vi "Transport_Reconnect.vi"(8 "error in (no error)":errorcluster={"status"=FALSE, "code"=0, "source"="\"\""}, 10 "reconnection policy":string, 11 "Channel refs":string) -> (0 "error out":errorcluster={"status"=FALSE, "code"=0, "source"="\"\""}, 2 "status ok":bool, 3 "New connection or failure":string)   [LabVIEW 2026]
doc: "INTENT: Recover non-running communication session. LOGIC: Tear down broken refs, negotiate capabilities, reconcile run identity and report outstanding status."
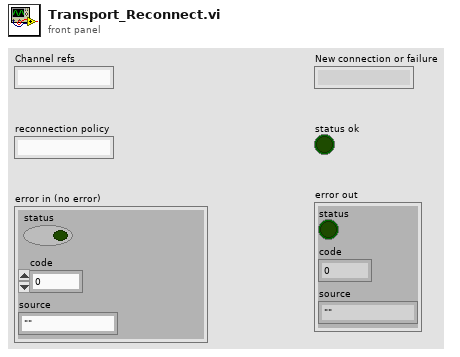
[diagram p1: front panel]
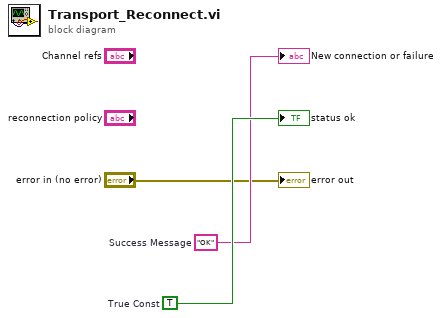
[diagram p0: block diagram]
diagram:
  w3 = TRUE  # True Const
  w2 = "OK"  # Success Message
  "New connection or failure" <- w2
  "status ok" <- w3
  "error out" <- "error in (no error)"
